vi "Front Panel JPEG file converter.vi"(8 "error in":errorcluster, 10 "JPEG file name":path, 11 "VI Path":path) -> (0 "error out":errorcluster)   [LabVIEW 2018]
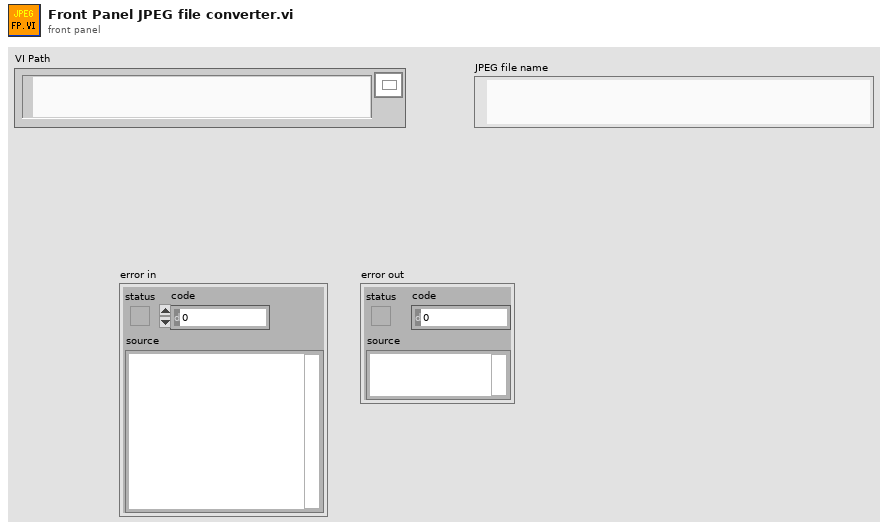
[diagram p1: front panel]
types:
  T1 = typedef "imagedata.ctl" = cluster{"image type":i32, "image depth":i32, "image":u8[], "mask":u8[], "colors":u32[], "Rectangle":cluster{"left":i16, "top":i16, "right":i16, "bottom":i16}}
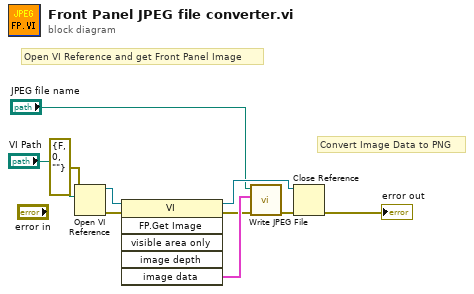
[diagram p0: block diagram]
diagram:
  # "Convert Image Data to PNG"
  # "Open VI Reference and get Front Panel Image"
  n1 = Open VI Reference(vi path="VI Path", error in (no error)=errorcluster {"status"=FALSE, "code"=0, "source"=""}) -> (vi reference=w10:refnum<vi>, error out=w9:errorcluster)  [unwired: 4 in]
  n2 = invoke class="VI" method="FP.Get Image"(reference=w10, error in=w9) -> (reference out=w8:refnum<vi>, error out=w5:errorcluster, "image data"=w6:T1)  [unwired: 4 in, 3 out]
  n3 = call <vilib>:"Write JPEG File.vi"("error in (no error)"=w5, "image data"=w6, "path to JPEG file"="JPEG file name") -> ("error out"=w3:errorcluster)  [unwired: 7 in, 1 out]
  n4 = Close Reference(reference=w8, error in (no error)=w3) -> (error out=→"error out":errorcluster)
